vi "Set Turn Table Target Angle and Go.vi"(8 "error in (no error)":errorcluster, 10 "Target Angle":dbl, 11 "VISA Refnum in":refnum<visa-resource-name>) -> (0 "error out":errorcluster, 3 "VISA Refnum out":refnum<visa-resource-name>)   [LabVIEW 2023, in "Turn Table and Mast.lvlib" / "ETS_EM2090.lvclass"]
uses:
  ETS_EM2090.lvclass
  ETS_EM2090.lvclass/ETS_EM2090.ctl
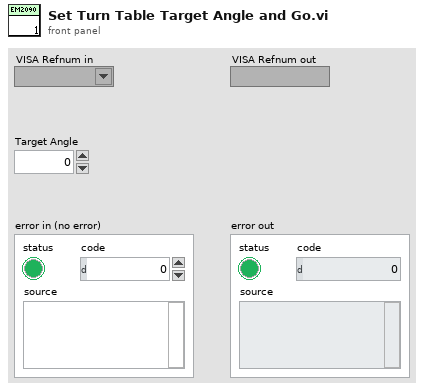
[diagram p1: front panel]
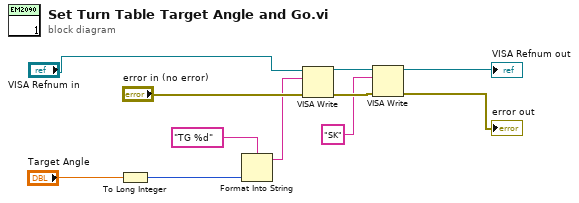
[diagram p0: block diagram]
diagram:
  n1 = To Long Integer(number="Target Angle") -> (32bit integer=w1:i32)
  n2 = Format Into String(format string="TG %d" ("포맷 문자열"), w1) -> (resulting string=w7:string)  [unwired: 2 in, 1 out]
  n3 = VISA Write(VISA resource name="VISA Refnum in", write buffer=w7, error in (no error)="error in (no error)") -> (VISA resource name out=w6:refnum<visa-resource-name>, error out=w5:errorcluster)  [unwired: 1 out]
  n4 = VISA Write(VISA resource name=w6, write buffer="SK" ("포맷 문자열"), error in (no error)=w5) -> (VISA resource name out=→"VISA Refnum out":refnum<visa-resource-name>, error out=→"error out":errorcluster)  [unwired: 1 out]
